vi "Signal Assembly Result Cluster.vi"(8 "Right Read MIN":i32, 9 "AR BN#":i32[](array[numeric]), 10 "Long Signal#":i32, 11 "AR T#":i32) -> (0 "RR MIN Over S#":i32, 3 "Total assembly C":T1 {"Assembly Ratio 2" format="%#_3g"; "Assembly Ratio" format="%#_3g"})   [LabVIEW 2018]
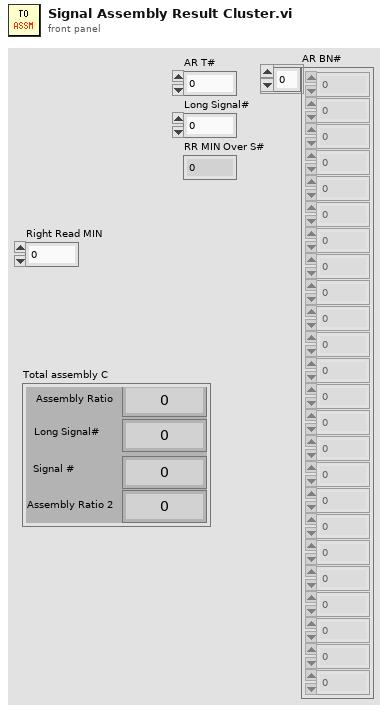
[diagram p1: front panel]
types:
  T1 = cluster{"Assembly Ratio":dbl, "Long Signal#":i32, "Signal #":i32, "Assembly Ratio 2":dbl}
  T2 = cluster{dbl, "Long Signal#":i32, "AR T#":i32, dbl}
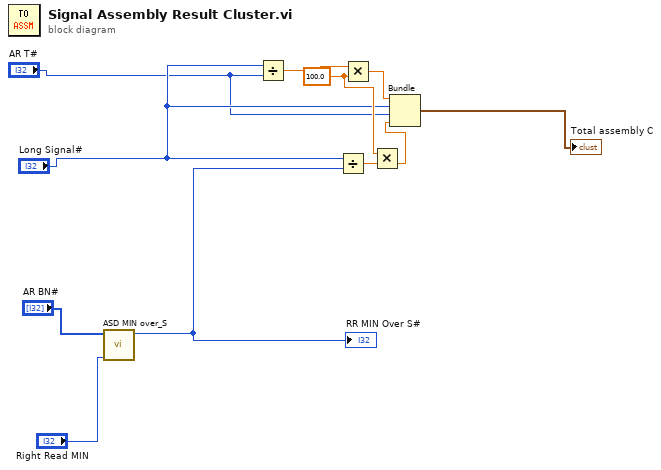
[diagram p0: block diagram]
diagram:
  w7 = 100.0 ("y")
  n1 = call "ASD MIN over_S.vi"("Right Read MIN"="Right Read MIN", "AR BN#"="AR BN#") -> ("RR MIN Over S#"=w1:i32)  [unwired: 9 in]
  "RR MIN Over S#" <- w1
  n2 = Divide(x="Long Signal#", y="AR T#") -> (x/y=w11:dbl)
  n3 = Divide(x="Long Signal#", y=w1) -> (x/y=w9:dbl)
  n4 = Multiply(x=w11, y=w7) -> (x*y=w10:dbl)
  n5 = Multiply(x=w7, y=w9) -> (x*y=w8:dbl)
  n6 = Bundle(w10, "Long Signal#"="Long Signal#", "AR T#"="AR T#", w8) -> (→"Total assembly C":T2)  [unwired: 1 in]
